vi "Make Message.vi"(8 "error in (no error)":errorcluster, 9 "Message Type":T1, 10 "Method Qualified Name":string, 11 "Message Maker in":refnum<class "Message Maker.lvclass">) -> (0 "error out":errorcluster, 3 "Message Maker out":refnum<class "Message Maker.lvclass">)   [LabVIEW 2023, in "Message Maker.lvclass"]
doc: "Builds a message for the method specified\n\nAuthor: Derek Trepanier\nCopyright: MGI 2015"
uses:
  Message Maker.lvclass
  Message Type.ctl
  Message Status.ctl
  Message Maker.lvclass/Message Maker.ctl
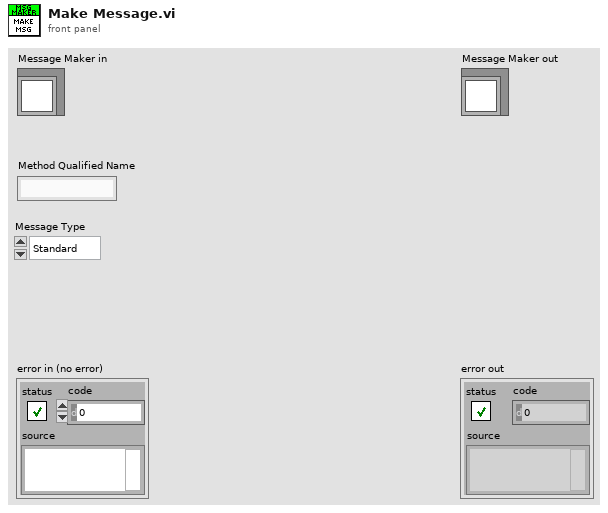
[diagram p1: front panel]
types:
  T1 = typedef "Message Maker.lvclass/Message Type.ctl" = enum16{"Standard", "Async"}
  T2 = typedef "Message Maker.lvclass/Message Status.ctl" = enum16{"Message Not Created", "Message Out of Date", "Message OK", "Never update"}
  T3 = typedef "Message Maker.lvclass/Message Recipient Type.ctl" = enum16{"Actor", "Interface", "Async Actor"}
  T4 = typedef "Message Maker.lvclass/Scripting Refs.ctl" = cluster{"Actor Method VI":refnum<vi>, "Actor Class":refnum<vi>, "Message Class":refnum<vi>}
  T5 = typedef "Message Maker.lvclass/Wiring Spec.ctl" = cluster{"Actor":cluster{"In":i32, "Out":i32}, "Error":cluster{"In":i32, "Out":i32}, "Terminals":cluster{"Position":T6, "Terminal":i32}[]}
  T6 = typedef "Message Maker.lvclass/Connector Pane Position.ctl" = enum16{"Left", "Top", "Bottom", "Right"}
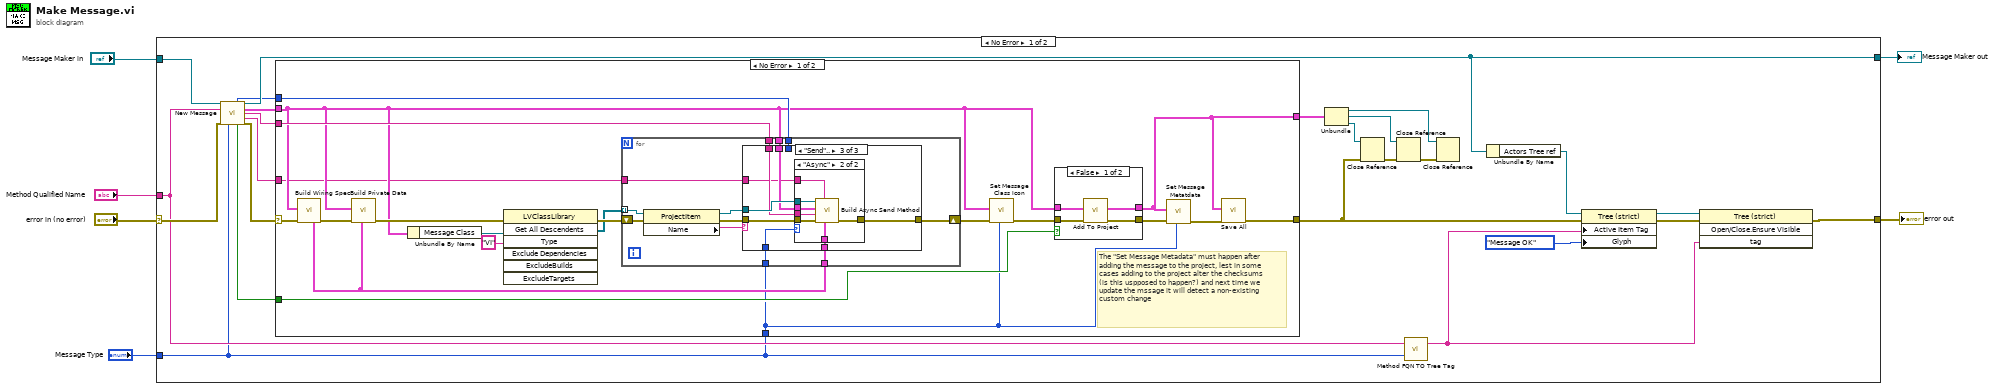
[diagram p0: block diagram]
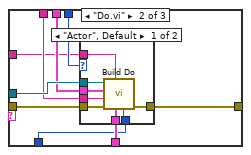
[diagram p4: hidden frame]
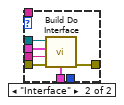
[diagram p5: hidden frame]
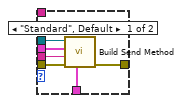
[diagram p6: hidden frame]
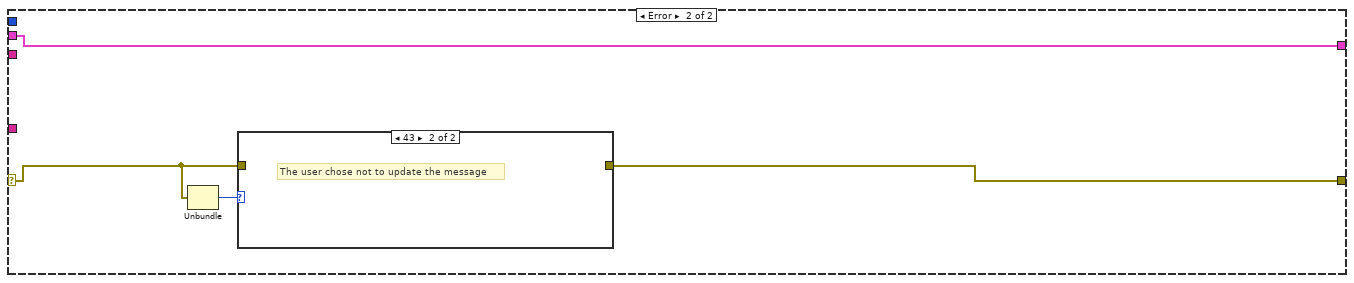
[diagram p7: hidden frame]
diagram:
  n1 = case shown="No Error" "error in (no error)" {
    selector: "error in (no error)" -> [w30 w120]
    tunnel: [w13 w120] -> w5
    tunnel: [w19 w119] -> w3
    tunnel: "Message Maker in" -> [w29 w119]
    tunnel: "Method Qualified Name" -> [w10 _]
    tunnel: "Message Type" -> [w8 _]
    frame No Error {
      n2 = call "New Message.vi"("Message Maker in"=w29, "Method Qualified Name"=w10, "error in (no error)"=w30, "Message Type"=w8) -> ("Message Recipient Type"=w11:T3, "Message Maker out"=w19:refnum<class "Message Maker.lvclass">, "References"=w24:T4, "AF Library FQN"=w12:string, "Async AF Library FQN"=w7:string, "Updating?"=w25:bool, "error out"=w20:errorcluster)  [unwired: 5 in]
      n3 = case shown="No Error" w20 {
        selector: w20 -> [w34 w115]
        tunnel: w25 -> [w43 _]
        tunnel: w24 -> [w37 w117]
        tunnel: [w42 w114] -> w17
        tunnel: [w36 w117] -> w21
        tunnel: w12 -> [w40 _]
        tunnel: w11 -> [w39 _]
        tunnel: w8 -> [w31 _]
        tunnel: w7 -> [w35 _]
        frame No Error {
          # "The \"Set Message Metadata\" must happen after adding the message to the project, lest in some cases adding to the project alter the checksums (is this uspposed to happen?) and next time we update the mssage it will detect a non-existing custom change"
          n4 = call "Build Wiring Spec.vi"("error in (no error)"=w34, "References"=w37) -> ("error out"=w50:errorcluster, "Wiring Spec"=w45:T5)  [unwired: 8 in]
          n5 = call "Build Private Data.vi"("Wiring Spec"=w45, "error in (no error)"=w50, "References"=w37) -> ("error out"=w46:errorcluster)  [unwired: 8 in]
          n6 = Unbundle By Name(w37) -> ("Message Class"=w44:refnum<vi>)
          n7 = invoke class="LVClassLibrary" method="Get All Descendents"(reference=w44, error in=w46, "Type"="VI") -> (error out=w49:errorcluster, "All Descendents"=w48:refnum<vi>[])  [unwired: 4 in, 5 out]
          n8 = for {
            tunnel: w48 -> [w68] mode=indexing
            shift-right: [w63] -> w41
            shift-left: w49 -> [w65]
            tunnel: w37 -> [w62]
            tunnel: w45 -> [w61]
            tunnel: w40 -> [w60]
            tunnel: w39 -> [w59]
            tunnel: w31 -> [w58]
            tunnel: w35 -> [w57]
            n9 = property class="ProjectItem"(reference=w68, error in=w65) -> (reference out=w66:refnum<vi>, error out=w64:errorcluster, "Name"=w67:string)
            n10 = case shown="\"Send\".." w67 {
              tunnel: w66 -> [_ w78 w100]
              tunnel: w64 -> [w69 w77 w98]
              tunnel: [w69 w76 w99] -> w63
              tunnel: w62 -> [_ w74 w97]
              tunnel: w61 -> [_ w75 w96]
              tunnel: w60 -> [_ w73 w95]
              tunnel: w59 -> [_ w72 _]
              tunnel: w58 -> [_ w71 w94]
              tunnel: w57 -> [_ w70 w93]
              frame Default {
              }
              frame "Do.vi" {
                n11 = case shown="\"Actor\", Default" w72 {
                  tunnel: w78 -> [w86 w90]
                  tunnel: w77 -> [w85 w92]
                  tunnel: [w84 w91] -> w76
                  tunnel: w75 -> [w83 w87]
                  tunnel: w74 -> [w82 w89]
                  tunnel: w73 -> [w81 w88]
                  tunnel: w71 -> [w80 _]
                  tunnel: w70 -> [w79 _]
                  frame "Actor", Default {
                    n12 = call "Build Do.vi"("Message Type"=w80, "Wiring Spec"=w83, "Async AF Library FQN"=w79, "error in (no error)"=w85, "AF Library FQN"=w81, "References"=w82, "Do VI"=w86) -> ("error out"=w84:errorcluster)  [unwired: 4 in]
                  }
                  frame "Interface" {
                    n13 = call "Build Do Interface.vi"("Wiring Spec"=w87, "error in (no error)"=w92, "AF Library FQN"=w88, "References"=w89, "Do VI"=w90) -> ("error out"=w91:errorcluster)  [unwired: 6 in]
                  }
                }
              }
              frame "Send".. {
                n14 = case shown="\"Async\"" w94 {
                  tunnel: w100 -> [w106 w113]
                  tunnel: [w105 w107] -> w99
                  tunnel: w98 -> [w104 w112]
                  tunnel: w97 -> [w103 w111]
                  tunnel: w96 -> [w102 w110]
                  tunnel: w95 -> [w101 w109]
                  tunnel: w93 -> [_ w108]
                  frame "Standard", Default {
                    n15 = call "Build Send Method.vi"("Wiring Spec"=w102, "error in (no error)"=w104, "AF Library FQN"=w101, "References"=w103, "Send VI"=w106) -> ("error out"=w105:errorcluster)  [unwired: 6 in]
                  }
                  frame "Async" {
                    n16 = call "Build Async Send Method.vi"("Wiring Spec"=w110, "Async AF Library FQN"=w108, "error in (no error)"=w112, "AF Library FQN"=w109, "References"=w111, "Send VI"=w113) -> ("error out"=w107:errorcluster)  [unwired: 5 in]
                  }
                }
              }
            }
          }
          n17 = call "Set Message Class Icon.vi"("Message Type"=w31, "error in (no error)"=w41, "References"=w37) -> ("error out"=w33:errorcluster)  [unwired: 8 in]
          n18 = case shown="False" w43 {
            tunnel: w33 -> [w54 w56]
            tunnel: w37 -> [w53 w55]
            tunnel: [w52 w56] -> w32
            tunnel: [w51 w55] -> w36
            frame False {
              n19 = call "Add To Project.vi"("error in (no error)"=w54, "References"=w53) -> ("error out"=w52:errorcluster, "Out"=w51:T4)  [unwired: 8 in]
            }
            frame True {
            }
          }
          n20 = call "Set Message Metatdata.vi"("Message Type"=w31, "error in (no error)"=w32, "References"=w36) -> ("error out"=w38:errorcluster)  [unwired: 8 in]
          n21 = call "Save All.vi"("error in (no error)"=w38, "References"=w36) -> ("error out"=w42:errorcluster)  [unwired: 9 in]
        }
        frame Error {
          n22 = Unbundle(w115) -> ("code"=w116:i32)  [unwired: 2 out]
          n23 = case shown="43" w116 {
            tunnel: w115 -> [w118 _]
            tunnel: [w118 _] -> w114
            frame 0, Default {
            }
            frame 43 {
              # "The user chose not to update the message"
            }
          }
        }
      }
      n24 = Unbundle(w21) -> ("Actor Method VI"=w28:refnum<vi>, "Actor Class"=w27:refnum<vi>, "Message Class"=w26:refnum<vi>)
      n25 = Close Reference(reference=w26, error in (no error)=w17) -> (error out=w22:errorcluster)
      n26 = Close Reference(reference=w27, error in (no error)=w22) -> (error out=w23:errorcluster)
      n27 = call "Method FQN TO Tree Tag.vi"("Message Type"=w8, "Method FQN"=w10) -> ("Method Tree Tag"=w9:string)  [unwired: 1 in]
      n28 = Close Reference(reference=w28, error in (no error)=w23) -> ()  [unwired: 1 out]
      n29 = Unbundle By Name(w19) -> ("Actors Tree ref"=w18:refnum<vi>)
      n30 = property class="Tree (strict)"(reference=w18, error in=w17, "Active Item Tag"=w9, "Glyph"=Message_Status."Message OK" ("Message Status")) -> (reference out=w15:refnum<vi>, error out=w14:errorcluster)
      n31 = invoke class="Tree (strict)" method="Open/Close.Ensure Visible"(reference=w15, error in=w14, "tag"=w9) -> (error out=w13:errorcluster)  [unwired: 1 in, 3 out]
    }
    frame Error {
    }
  }
  "error out" <- w5
  "Message Maker out" <- w3
